vi "Measurement UI.vi"() -> ()   [LabVIEW 2021, in "Efficiency And Load Regulation_PMIC.lvlib"]
uses:
  Efficiency And Load Regulation_PMIC.lvlib
panel:
  in  "MeasGraphs":T1(tab)
  out "EfficiencyGraph":T2(graph)
  out "LoadRegulationGraph(V/A)":T2(graph)
  out "LoadRegulationGraph(%)":T2(graph)
  out "Maximum load regulation":dbl[](array[numeric])
  out "Minimum load regulation":dbl[](array[numeric])
  out "Maximum load voltage":dbl[](array[numeric])
  out "Minimum load voltage":dbl[](array[numeric])
  out "Maximum efficiency":dbl[](array[numeric])
  out "Minimum efficiency":dbl[](array[numeric])
  out "Source sweep points":i32
  out "Load voltage deviation":dbl[](array[numeric])
  out "Load voltages":dbl[](array[numeric])
  out "Voltage values":dbl[](array[numeric])
  out "Load sweep points":i32
  out "Efficiency":dbl[](array[numeric])
  out "Load currents":dbl[](array[numeric])
  in  "Source resource name":string caption="RESOURCE NAME"
  in  "Load resource name":string caption="RESOURCE NAME"
  out "MeasTable":string[][](table)
  in  "Measurement timeout":dbl=10.0 caption="MEASUREMENT TIME-OUT" format="%#_6ps"
  in  "Load sense":i32(ring)=1009 caption="SENSE" items=["Local"=1008, "Remote"=1009]
  in  "Source sense":i32(ring)=1009 caption="SENSE" items=["Local"=1008, "Remote"=1009]
  out "Status":string
  in  "ELOADResourceName":refnum<k15> caption="RESOURCE NAME"
  in  "PPSResourceName":refnum<k15> caption="RESOURCE NAME"
  in  "Load sweep type":string(combo)="Logarithmic" caption="SWEEP TYPE"
  in  "DUT setup time":dbl=1.0 caption="DUT SETUP TIME" format="%#_6ps"
  in  "Source stop voltage":dbl=20.0 caption="STOP VOLTAGE" format="%#_6pV"
  in  "Source start voltage":dbl=6.0 caption="START VOLTAGE" format="%#_6pV"
  in  "Source voltage sweep points":i32=4 caption="NO. OF POINTS"
  in  "Aperture time":dbl=0.005 caption="APERTURE TIME" format="%#_6ps"
  in  "Source delay":dbl=0.005 caption="SOURCE DELAY" format="%#_6ps"
  in  "Load current sweep points/points per decade":i32=10 caption="PTS/PTS PER DECADE"
  in  "Load stop current":dbl=24.0 caption="STOP CURRENT" format="%#_6pA"
  in  "Load start current":dbl=0.1 caption="START CURRENT" format="%#_6pA"
  in  "Load voltage limit range":dbl=6.0 caption="VOLTAGE LIMIT RANGE" format="%#_6pV"
  in  "Source current limit":dbl=25.0 caption="CURRENT LIMIT" format="%#_6pA"
  in  "Source maximum power":dbl=300.0 caption="MAXIMUM POWER" format="%#_6pW"
  in  "Load configuration":string="Load configuration"
  in  "Source configuration":string="Source configuration"
  in  "Measurement settings":string="Measurement settings"
  in  "Nominal output voltage":dbl=3.3 caption="NOMINAL OUTPUT VOLTAGE" format="%#_6pV"
  in  "Mode of operation":T3(ring)=enum."Perform measurement" caption="MODE OF OPERATION"
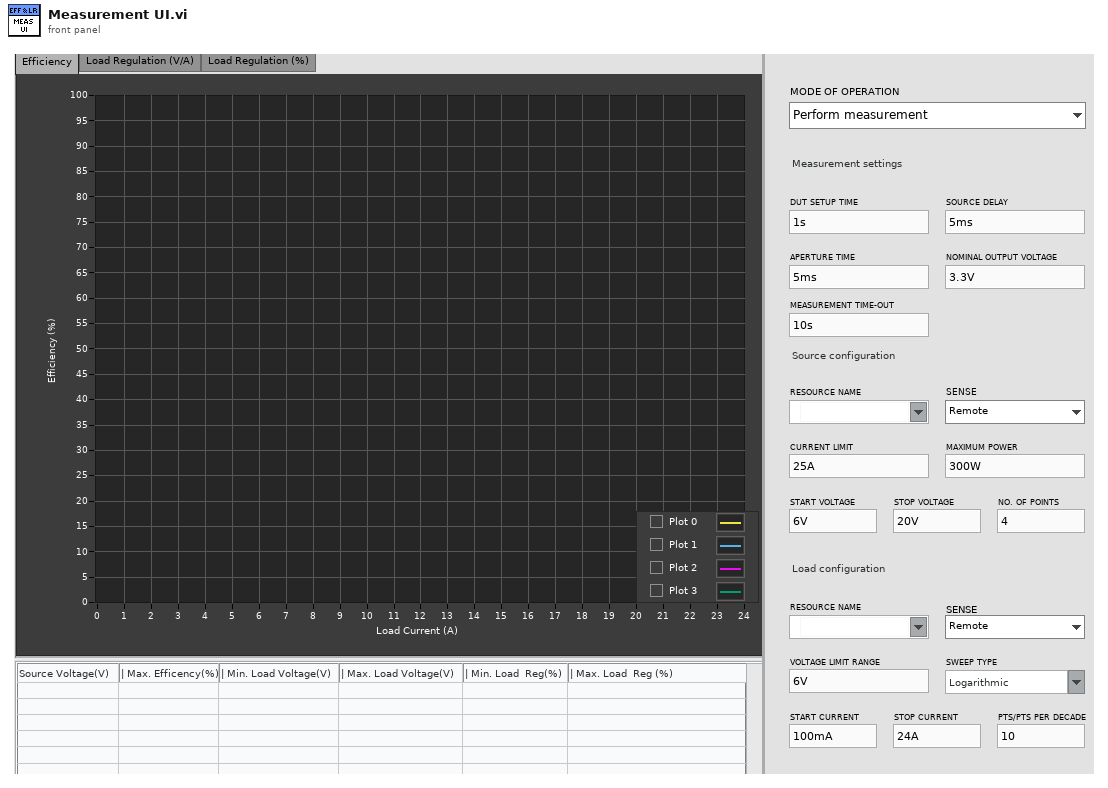
[diagram p1: front panel]
types:
  T1 = enum32{"Efficiency", "Load Regulation (V/A)", "Load Regulation (%)", "Hidden Controls"}
  T2 = cluster{"Load currents":dbl[], "Efficiency":dbl[]}[]
  T3 = enum32{"Power on the DUT", "Perform measurement", "Power off the DUT"}
  T4 = cluster{"Load currents":dbl[], "Efficiency":dbl[]}
  T5 = cluster{"Load currents":dbl[], "Load voltages":dbl[]}
  T6 = cluster{"Load currents":dbl[], "Load voltage deviation":dbl[]}
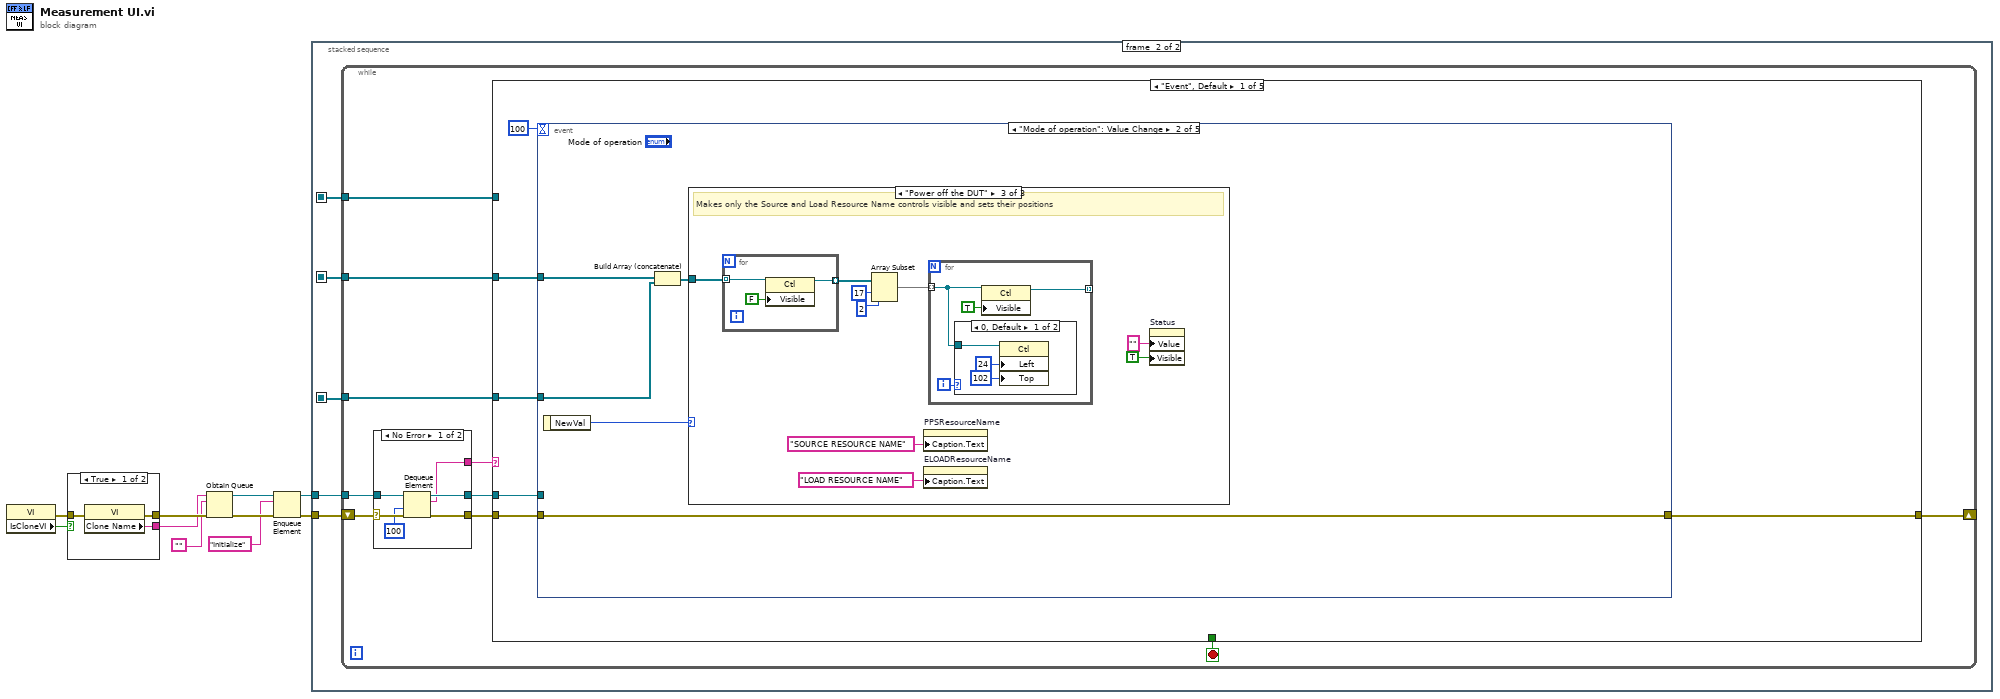
[diagram p0: block diagram]
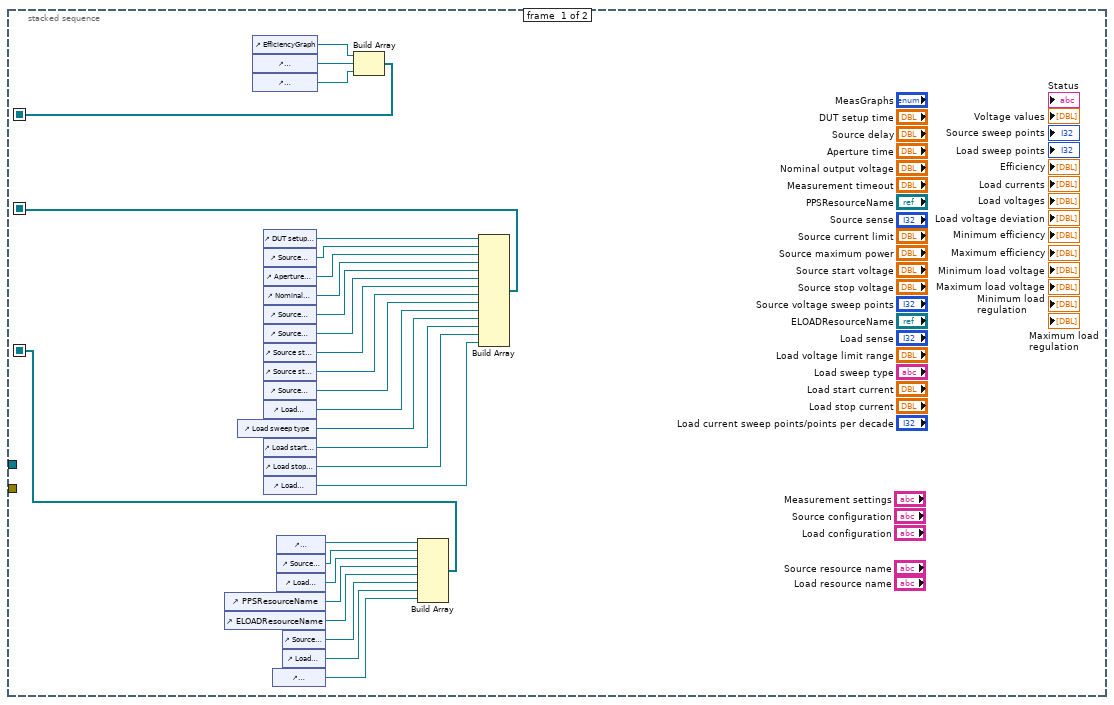
[diagram p2: hidden frame]
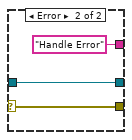
[diagram p3: hidden frame]
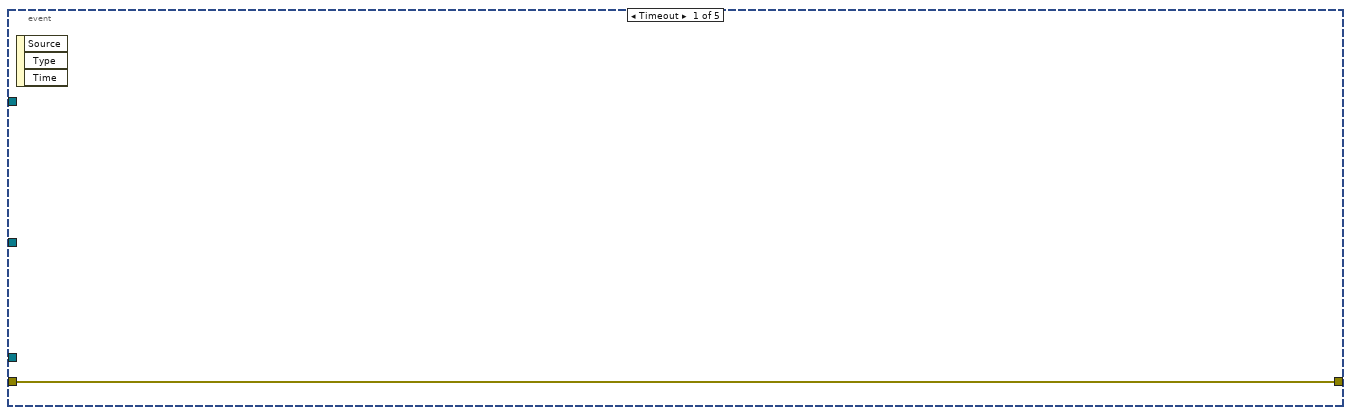
[diagram p4: hidden frame]
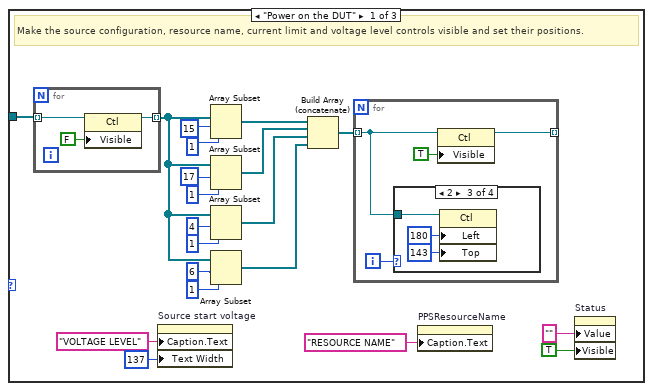
[diagram p5: hidden frame]
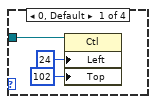
[diagram p6: hidden frame]
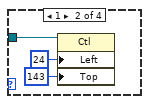
[diagram p7: hidden frame]
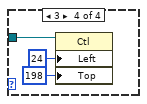
[diagram p8: hidden frame]
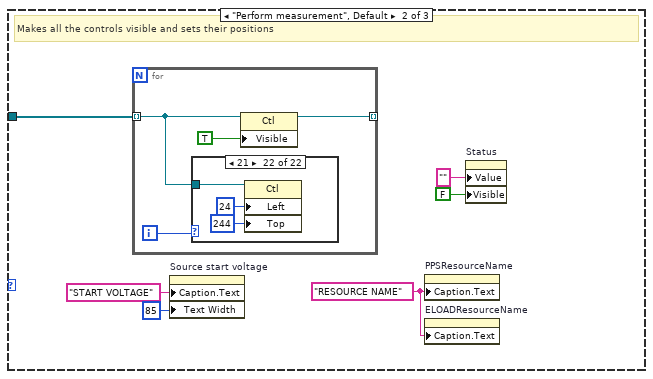
[diagram p9: hidden frame]
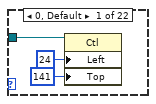
[diagram p10: hidden frame]
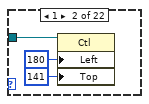
[diagram p11: hidden frame]
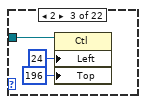
[diagram p12: hidden frame]
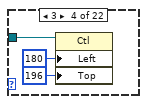
[diagram p13: hidden frame]
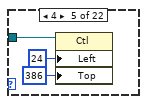
[diagram p14: hidden frame]
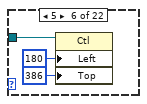
[diagram p15: hidden frame]
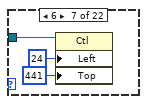
[diagram p16: hidden frame]
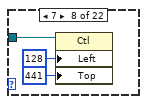
[diagram p17: hidden frame]
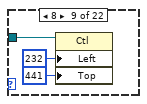
[diagram p18: hidden frame]
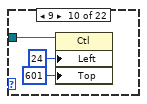
[diagram p19: hidden frame]
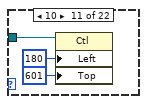
[diagram p20: hidden frame]
diagram:
  n1 = property class="VI"() -> (error out=w1:errorcluster, "IsCloneVI"=w2:bool)  [unwired: 2 in, 1 out]
  n2 = case shown="True" w2 {
    tunnel: [w13 w16] -> w10
    tunnel: [w12 w15] -> w9
    tunnel: w1 -> [w11 w14]
    frame True {
      n3 = property class="VI"(error in=w11) -> (error out=w13:errorcluster, "Clone Name"=w12:string)  [unwired: 1 in, 1 out]
    }
    frame False {
      n4 = property class="VI"(error in=w14) -> (error out=w16:errorcluster, "Name"=w15:string)  [unwired: 1 in, 1 out]
    }
  }
  n5 = Obtain Queue(name (unnamed)=w9, element data type="", error in (no error)=w10) -> (queue out=w6:refnum<queue>, error out=w8:errorcluster)  [unwired: 2 in, 1 out]
  n6 = Enqueue Element(queue=w6, element="Initialize", error in (no error)=w8) -> (queue out=w5:refnum<queue>, error out=w7:errorcluster)  [unwired: 1 in, 1 out]
  n7 = stacked-sequence {
    seq-local: [w20 _] -> [_ w47]
    seq-local: [w21 _] -> [_ w46]
    seq-local: [w22 _] -> [_ w45]
    tunnel: w7 -> [_ w49]
    tunnel: w5 -> [_ w48]
    frame #0 {
      n8 = control-ref of="PPSResourceName"() -> (w27:refnum<vi>)
      n9 = control-ref of="ELOADResourceName"() -> (w26:refnum<vi>)
      n10 = control-ref of="Load sweep type"() -> (w35:refnum<vi>)
      n11 = control-ref of="EfficiencyGraph"() -> (w25:refnum<vi>)
      n12 = control-ref of="LoadRegulationGraph(V/A)"() -> (w24:refnum<vi>)
      n13 = control-ref of="LoadRegulationGraph(%)"() -> (w23:refnum<vi>)
      n14 = control-ref of="DUT setup time"() -> (w44:refnum<vi>)
      n15 = control-ref of="Source delay"() -> (w43:refnum<vi>)
      n16 = control-ref of="Aperture time"() -> (w42:refnum<vi>)
      n17 = control-ref of="Nominal output voltage"() -> (w31:refnum<vi>)
      n18 = control-ref of="Source current limit"() -> (w41:refnum<vi>)
      n19 = control-ref of="Source maximum power"() -> (w40:refnum<vi>)
      n20 = control-ref of="Source start voltage"() -> (w39:refnum<vi>)
      n21 = control-ref of="Source stop voltage"() -> (w38:refnum<vi>)
      n22 = control-ref of="Source voltage sweep points"() -> (w37:refnum<vi>)
      n23 = control-ref of="Load voltage limit range"() -> (w36:refnum<vi>)
      n24 = control-ref of="Load start current"() -> (w34:refnum<vi>)
      n25 = control-ref of="Load stop current"() -> (w33:refnum<vi>)
      n26 = control-ref of="Load current sweep points/points per decade"() -> (w32:refnum<vi>)
      n27 = control-ref of="Measurement timeout"() -> (w17:refnum<vi>)
      n28 = control-ref of="Measurement settings"() -> (w30:refnum<vi>)
      n29 = control-ref of="Source configuration"() -> (w28:refnum<vi>)
      n30 = control-ref of="Load configuration"() -> (w29:refnum<vi>)
      n31 = control-ref of="Source sense"() -> (w19:refnum<vi>)
      n32 = control-ref of="Load sense"() -> (w18:refnum<vi>)
      n33 = Build Array(w25, w24, w23) -> (w20:refnum<vi>[])
      n34 = Build Array(w30, w28, w29, w27, w26, w19, w18, w17) -> (w22:refnum<vi>[])
      n35 = Build Array(w44, w43, w42, w31, w41, w40, w39, w38, w37, w36, w35, w34, w33, w32) -> (w21:refnum<vi>[])
    }
    frame #1 {
      n36 = while {
        shift-right: [w54] -> _
        shift-left: w49 -> [w59]
        tunnel: w48 -> [w57]
        tunnel: w46 -> [w52]
        tunnel: w45 -> [w51]
        tunnel: w47 -> [w50]
        stop <- w53 stop-if-true
        n37 = case shown="No Error" w59 {
          selector: w59 -> [w65 w68]
          tunnel: [w64 w68] -> w58
          tunnel: w57 -> [w63 w67]
          tunnel: [w62 w67] -> w56
          tunnel: [w61 "Handle Error"] -> w55
          frame No Error {
            n38 = Dequeue Element(queue=w63, timeout in ms (-1)=100, error in (no error)=w65) -> (queue out=w62:refnum<queue>, element=w61:string, error out=w64:errorcluster)  [unwired: 1 out]
          }
          frame Error {
          }
        }
        n39 = case shown="\"Event\", Default" w55 {
          tunnel: w58 -> [w73 w230 w253 w331 w332]
          tunnel: w56 -> [w71 _ _ w329 _]
          tunnel: [w74 w230 w253 w323 w332] -> w54
          tunnel: [_ _ _ TRUE _] -> w53
          tunnel: w52 -> [w70 _ _ w321 _]
          tunnel: w51 -> [w69 _ _ w320 _]
          tunnel: w50 -> [_ w229 w243 w322 _]
          frame "Event", Default {
            n40 = event shown="[1] \"Mode of operation\": Value Change" {
              selector: _ -> [_ _ _ _ _]
              dyn-events: _ -> [_ _ _ _ _]
              timeout: 100 -> [_ _ _ _ _]
              tunnel: [w75 w76 w218 w220 w224] -> w74
              tunnel: w73 -> [w75 w76 w218 w220 w225]
              tunnel: w71 -> [_ _ _ _ w223]
              tunnel: w70 -> [_ w77 _ _ _]
              tunnel: w69 -> [_ w79 _ _ _]
              event Timeout {
                n41 = event-data() -> ()  [unwired: 1 in, 3 out]
              }
              event "Mode of operation": Value Change {
                n42 = event-data() -> ("NewVal"=w80:T3)  [unwired: 1 in]
                n43 = Build Array (concatenate)(w77, w79) -> (w78:refnum<vi>[])
                n44 = case shown="\"Power off the DUT\"" w80 {
                  tunnel: w78 -> [w92 w125 w201]
                  frame "Power on the DUT" {
                    # "Make the source configuration, resource name, current limit and voltage level controls visible and set their positions."
                    n45 = for {
                      tunnel: w92 -> [w103] mode=indexing
                      tunnel: [w101] -> w89 mode=indexing
                      n46 = property class="Ctl"(reference=w103, "Visible"=FALSE) -> (reference out=w101:refnum<vi>)  [unwired: 1 in, 1 out]
                    }
                    n47 = property on="Source start voltage" class="DigNum (strict)"("Caption.Text"="VOLTAGE LEVEL", "Text Width"=u32 137) -> ()  [unwired: 2 in, 2 out]
                    n48 = Array Subset(array=w89, index=15 ("length"), length=1 ("index")) -> (w91:refnum<vi>[])
                    n49 = Array Subset(array=w89, index=17 ("length"), length=1 ("index")) -> (w90:refnum<vi>[])
                    n50 = Array Subset(array=w89, index=4 ("length"), length=1 ("index")) -> (w88:refnum<vi>[])
                    n51 = Array Subset(array=w89, index=6 ("length"), length=1 ("index")) -> (w86:refnum<vi>[])
                    n52 = Build Array (concatenate)(w91, w90, w88, w86) -> (w87:refnum<vi>[])
                    n53 = for {
                      tunnel: [w106] -> _ mode=indexing
                      tunnel: w87 -> [w104] mode=indexing
                      i -> [w105]
                      n54 = case shown="2" w105 {
                        tunnel: w104 -> [w110 w113 w116 w119]
                        frame 0, Default {
                          n55 = property class="Ctl"(reference=w110, "Left"=24 ("Position:Left"), "Top"=102 ("Position:Top")) -> ()  [unwired: 1 in, 2 out]
                        }
                        frame 1 {
                          n56 = property class="Ctl"(reference=w113, "Left"=24 ("Position:Left"), "Top"=143 ("Position:Top")) -> ()  [unwired: 1 in, 2 out]
                        }
                        frame 2 {
                          n57 = property class="Ctl"(reference=w116, "Left"=180 ("Position:Left"), "Top"=143 ("Position:Top")) -> ()  [unwired: 1 in, 2 out]
                        }
                        frame 3 {
                          n58 = property class="Ctl"(reference=w119, "Left"=24 ("Position:Left"), "Top"=198 ("Position:Top")) -> ()  [unwired: 1 in, 2 out]
                        }
                      }
                      n59 = property class="Ctl"(reference=w104, "Visible"=TRUE) -> (reference out=w106:refnum<vi>)  [unwired: 1 in, 1 out]
                    }
                    n60 = property on="PPSResourceName" class="IVIName"("Caption.Text"="RESOURCE NAME") -> ()  [unwired: 2 in, 2 out]
                    n61 = property on="Status" class="Str"("Value"="" ("Status"), "Visible"=TRUE) -> ()  [unwired: 2 in, 2 out]
                  }
                  frame "Perform measurement", Default {
                    w123 = "RESOURCE NAME" ("Caption.Text")
                    # "Makes all the controls visible and sets their positions"
                    n62 = for {
                      tunnel: w125 -> [w126] mode=indexing
                      tunnel: [w128] -> _ mode=indexing
                      i -> [w127]
                      n63 = case shown="21" w127 {
                        tunnel: w126 -> [w132 w135 w138 w141 w144 w147 w150 w153 w156 w159 w162 w165 w168 w171 w174 w177 w180 w183 w186 w187 w190 w193]
                        frame 0, Default {
                          n64 = property class="Ctl"(reference=w132, "Left"=24 ("Position:Left"), "Top"=141 ("Position:Top")) -> ()  [unwired: 1 in, 2 out]
                        }
                        frame 1 {
                          n65 = property class="Ctl"(reference=w135, "Left"=180 ("Position:Left"), "Top"=141 ("Position:Top")) -> ()  [unwired: 1 in, 2 out]
                        }
                        frame 2 {
                          n66 = property class="Ctl"(reference=w138, "Left"=24 ("Position:Left"), "Top"=196 ("Position:Top")) -> ()  [unwired: 1 in, 2 out]
                        }
                        frame 3 {
                          n67 = property class="Ctl"(reference=w141, "Left"=180 ("Position:Left"), "Top"=196 ("Position:Top")) -> ()  [unwired: 1 in, 2 out]
                        }
                        frame 4 {
                          n68 = property class="Ctl"(reference=w144, "Left"=24 ("Position:Left"), "Top"=386 ("Position:Top")) -> ()  [unwired: 1 in, 2 out]
                        }
                        frame 5 {
                          n69 = property class="Ctl"(reference=w147, "Left"=180 ("Position:Left"), "Top"=386 ("Position:Top")) -> ()  [unwired: 1 in, 2 out]
                        }
                        frame 6 {
                          n70 = property class="Ctl"(reference=w150, "Left"=24 ("Position:Left"), "Top"=441 ("Position:Top")) -> ()  [unwired: 1 in, 2 out]
                        }
                        frame 7 {
                          n71 = property class="Ctl"(reference=w153, "Left"=128 ("Position:Left"), "Top"=441 ("Position:Top")) -> ()  [unwired: 1 in, 2 out]
                        }
                        frame 8 {
                          n72 = property class="Ctl"(reference=w156, "Left"=232 ("Position:Left"), "Top"=441 ("Position:Top")) -> ()  [unwired: 1 in, 2 out]
                        }
                        frame 9 {
                          n73 = property class="Ctl"(reference=w159, "Left"=24 ("Position:Left"), "Top"=601 ("Position:Top")) -> ()  [unwired: 1 in, 2 out]
                        }
                        frame 10 {
                          n74 = property class="Ctl"(reference=w162, "Left"=180 ("Position:Left"), "Top"=601 ("Position:Top")) -> ()  [unwired: 1 in, 2 out]
                        }
                        frame 11 {
                          n75 = property class="Ctl"(reference=w165, "Left"=24 ("Position:Left"), "Top"=656 ("Position:Top")) -> ()  [unwired: 1 in, 2 out]
                        }
                        frame 12 {
                          n76 = property class="Ctl"(reference=w168, "Left"=128 ("Position:Left"), "Top"=656 ("Position:Top")) -> ()  [unwired: 1 in, 2 out]
                        }
                        frame 13 {
                          n77 = property class="Ctl"(reference=w171, "Left"=232 ("Position:Left"), "Top"=656 ("Position:Top")) -> ()  [unwired: 1 in, 2 out]
                        }
                        frame 14 {
                          n78 = property class="Ctl"(reference=w174, "Left"=24 ("Position:Left"), "Top"=100 ("Position:Top")) -> ()  [unwired: 1 in, 2 out]
                        }
                        frame 15 {
                          n79 = property class="Ctl"(reference=w177, "Left"=24 ("Position:Left"), "Top"=292 ("Position:Top")) -> ()  [unwired: 1 in, 2 out]
                        }
                        frame 16 {
                          n80 = property class="Ctl"(reference=w180, "Left"=24 ("Position:Left"), "Top"=505 ("Position:Top")) -> ()  [unwired: 1 in, 2 out]
                        }
                        frame 17 {
                          n81 = property class="Ctl"(reference=w183, "Left"=24 ("Position:Left"), "Top"=331 ("Position:Top")) -> ()  [unwired: 1 in, 2 out]
                        }
                        frame 18 {
                          n82 = property class="Ctl"(reference=w186, "Left"=24 ("Position:Left"), "Top"=546 ("Position:Top")) -> ()  [unwired: 1 in, 2 out]
                        }
                        frame 19 {
                          n83 = property class="Ctl"(reference=w187, "Left"=180 ("Position:Left"), "Top"=331 ("Position:Top")) -> ()  [unwired: 1 in, 2 out]
                        }
                        frame 20 {
                          n84 = property class="Ctl"(reference=w190, "Left"=180 ("Position:Left"), "Top"=546 ("Position:Top")) -> ()  [unwired: 1 in, 2 out]
                        }
                        frame 21 {
                          n85 = property class="Ctl"(reference=w193, "Left"=24 ("Position:Left"), "Top"=244 ("Position:Top")) -> ()  [unwired: 1 in, 2 out]
                        }
                      }
                      n86 = property class="Ctl"(reference=w126, "Visible"=TRUE) -> (reference out=w128:refnum<vi>)  [unwired: 1 in, 1 out]
                    }
                    n87 = property on="Source start voltage" class="DigNum (strict)"("Caption.Text"="START VOLTAGE", "Text Width"=u32 85) -> ()  [unwired: 2 in, 2 out]
                    n88 = property on="PPSResourceName" class="IVIName"("Caption.Text"=w123) -> ()  [unwired: 2 in, 2 out]
                    n89 = property on="ELOADResourceName" class="IVIName"("Caption.Text"=w123) -> ()  [unwired: 2 in, 2 out]
                    n90 = property on="Status" class="Str"("Value"="" ("Status"), "Visible"=FALSE) -> ()  [unwired: 2 in, 2 out]
                  }
                  frame "Power off the DUT" {
                    # "Makes only the Source and Load Resource Name controls visible and sets their positions"
                    n91 = for {
                      tunnel: w201 -> [w206] mode=indexing
                      tunnel: [w205] -> w200 mode=indexing
                      n92 = property class="Ctl"(reference=w206, "Visible"=FALSE) -> (reference out=w205:refnum<vi>)  [unwired: 1 in, 1 out]
                    }
                    n93 = Array Subset(array=w200, index=17 ("length"), length=2 ("index")) -> (w202:refnum<vi>[])
                    n94 = property on="PPSResourceName" class="IVIName"("Caption.Text"="SOURCE RESOURCE NAME") -> ()  [unwired: 2 in, 2 out]
                    n95 = property on="ELOADResourceName" class="IVIName"("Caption.Text"="LOAD RESOURCE NAME") -> ()  [unwired: 2 in, 2 out]
                    n96 = for {
                      tunnel: w202 -> [w208] mode=indexing
                      tunnel: [w210] -> _ mode=indexing
                      i -> [w209]
                      n97 = case shown="0, Default" w209 {
                        tunnel: w208 -> [w214 w217]
                        frame 0, Default {
                          n98 = property class="Ctl"(reference=w214, "Left"=24 ("Position:Left"), "Top"=102 ("Position:Top")) -> ()  [unwired: 1 in, 2 out]
                        }
                        frame 1 {
                          n99 = property class="Ctl"(reference=w217, "Left"=24 ("Position:Left"), "Top"=157 ("Position:Top")) -> ()  [unwired: 1 in, 2 out]
                        }
                      }
                      n100 = property class="Ctl"(reference=w208, "Visible"=TRUE) -> (reference out=w210:refnum<vi>)  [unwired: 1 in, 1 out]
                    }
                    n101 = property on="Status" class="Str"("Value"="" ("Status"), "Visible"=TRUE) -> ()  [unwired: 2 in, 2 out]
                  }
                }
              }
              event "PPSResourceName": Value Change {
                n102 = event-data() -> ()  [unwired: 1 in, 1 out]
                n103 = property on="PPSResourceName" class="IVIName"() -> ("Value"=w219:refnum<k15>)  [unwired: 2 in, 2 out]
                n104 = property on="Source resource name" class="Str"("Value"=w219) -> ()  [unwired: 2 in, 2 out]
              }
              event "ELOADResourceName": Value Change {
                n105 = event-data() -> ()  [unwired: 1 in, 1 out]
                n106 = property on="ELOADResourceName" class="IVIName"() -> ("Value"=w221:refnum<k15>)  [unwired: 2 in, 2 out]
                n107 = property on="Load resource name" class="Str"("Value"=w221) -> ()  [unwired: 2 in, 2 out]
              }
              event Panel Close? {
                n108 = event-data() -> ()  [unwired: 1 in, 4 out]
                n109 = Enqueue Element(queue=w223, element="Exit", error in (no error)=w225) -> (error out=w224:errorcluster)  [unwired: 1 in, 2 out]
                n110 = event-data("Discard?"=TRUE) -> ()  [unwired: 1 in, 1 out]
              }
            }
          }
          frame "Initialize" {
            w228 = "<Select Device>"
            n111 = for {
              tunnel: w229 -> [w231] mode=indexing
              n112 = property class="XYGraph (strict)"(reference=w231, "ActPaletteTool"=2 ("Palette:Active Tool")) -> ()  [unwired: 1 in, 2 out]
            }
            n113 = property on="PPSResourceName" class="IVIName"("Value"=w228) -> ()  [unwired: 2 in, 2 out]
            n114 = property on="ELOADResourceName" class="IVIName"("Value"=w228) -> ()  [unwired: 2 in, 2 out]
            n115 = property on="Status" class="Str"("Visible"=FALSE) -> ()  [unwired: 2 in, 2 out]
          }
          frame "Post UI Update" {
            w242 = u32[] [15787074, 5682409, 15535092, 40563, 13983232, 35009, 15113984, 13400487, 15993633, 10221451, 8148942, 15869817, 32914, 10196480, 6271923, 16355671]  # Plot colors
            # "-Sets various properties of graphs like color, point style, plot name etc.\n-Increases the legend number of rows if the voltage values are less than 4 and \nif it is greater than 4 then make the default rows as 4 and enable the vertical scrollbar.\n-Also sets the plot minimum property to source sweep points which disables the unused plots in the graph."
            # "Plot the deleted array in the graph"
            # "This case will be triggered, after framework updates the User interface with result values."
            n116 = local read "Source sweep points"() -> (w241:i32)
            n117 = local read "Voltage values"() -> (w239:dbl[])
            n118 = for {
              tunnel: w239 -> [w273]
              tunnel: [w272] -> w240
              tunnel: w243 -> [w271] mode=indexing
              tunnel: w241 -> [w270]
              tunnel: w242 -> [w269]
              n119 = for {
                tunnel: w273 -> [w286] mode=indexing
                tunnel: [w286] -> w272 mode=indexing
                tunnel: w271 -> [w279]
                tunnel: w270 -> [w276]
                tunnel: w269 -> [w282] mode=indexing
                i -> [w280]
                n120 = Greater?(x=w280, y=3) -> (0:w284:bool)
                n121 = To Unsigned Long Integer(number=w280) -> (unsigned 32bit integer=w283:u32)
                n122 = Increment(x=w280) -> (x+1=w278:i32)
                n123 = Format Value(format string="%.3f", value (0)=w286) -> (output string=w289:string)  [unwired: 1 out]
                n124 = case shown="False" w284 {
                  tunnel: w279 -> [w295 w301]
                  tunnel: w278 -> [w294 _]
                  tunnel: [w293 w300] -> w277
                  tunnel: w276 -> [w291 w296]
                  tunnel: [w292 w299] -> w275
                  frame False {
                    n125 = property on="Property Node" class="XYGraph (strict)"(reference=w295, "LegScrollVis"=FALSE ("Legend:Scrollbar Visible"), "LegNumRows"=w294, "LegPlotMin"=w291) -> (reference out=w293:refnum<vi>, error out=w292:errorcluster)  [unwired: 1 in]
                  }
                  frame True {
                    n126 = property on="Property Node" class="XYGraph (strict)"(reference=w301, "LegScrollVis"=TRUE ("Legend:Scrollbar Visible"), "LegNumRows"=u32 4 ("Legend:Number of Rows"), "LegPlotMin"=w296) -> (reference out=w300:refnum<vi>, error out=w299:errorcluster)  [unwired: 1 in]
                  }
                }
                n127 = Concatenate Strings(" Vin = " ("string"), w289) -> (w274:string)
                n128 = property on="Property Node" class="XYGraph (strict)"(reference=w277, error in=w275, "Active Plot"=w283, "Plot.Point Style"=u8 5, "Plot.Plot Color"=w282, "Plot.Fill/Pt. Color"=w282, "Plot.Plot Name"=w274) -> ()  [unwired: 2 out]
              }
            }
            n129 = local read "Maximum load regulation"() -> (w234:dbl[])
            n130 = local read "Minimum load regulation"() -> (w235:dbl[])
            n131 = local read "Maximum load voltage"() -> (w236:dbl[])
            n132 = local read "Minimum load voltage"() -> (w237:dbl[])
            n133 = local read "Maximum efficiency"() -> (w238:dbl[])
            n134 = Array Size(array=w240) -> (size(s)=w250:i32)
            n135 = local read "Load voltage deviation"() -> (w252:dbl[])
            n136 = local read "Load sweep points"() -> (w247:i32)
            n137 = local read "Load voltages"() -> (w251:dbl[])
            n138 = local read "Load currents"() -> (w249:dbl[])
            n139 = local read "Efficiency"() -> (w248:dbl[])
            n140 = for {
              N: w250 -> [_]
              tunnel: [w318] -> w244 mode=indexing
              tunnel: [w317] -> w245 mode=indexing
              tunnel: [w316] -> w246 mode=indexing
              tunnel: w247 -> [w303]
              shift-right: [w311] -> _
              shift-left: w249 -> [w315]
              shift-right: [w309] -> _
              shift-left: w248 -> [w314]
              shift-right: [w308] -> _
              shift-left: w251 -> [w313]
              shift-right: [w307] -> _
              shift-left: w252 -> [w312]
              w302 = 0 ("index")
              n141 = Delete From Array(array=w315, length=w303, index=w302) -> (deleted portion=w310:dbl[], array with subset deleted=w311:dbl[])
              n142 = Delete From Array(array=w314, length=w303, index=w302) -> (deleted portion=w304:dbl[], array with subset deleted=w309:dbl[])
              n143 = Delete From Array(array=w313, length=w303, index=w302) -> (deleted portion=w305:dbl[], array with subset deleted=w308:dbl[])
              n144 = Delete From Array(array=w312, length=w303, index=w302) -> (deleted portion=w306:dbl[], array with subset deleted=w307:dbl[])
              n145 = Bundle("Load currents"=w310, "Efficiency"=w304) -> (w318:T4)  [unwired: 1 in]
              n146 = Bundle("Load currents"=w310, "Load voltages"=w305) -> (w317:T5)  [unwired: 1 in]
              n147 = Bundle("Load currents"=w310, "Load voltage deviation"=w306) -> (w316:T6)  [unwired: 1 in]
            }
            "EfficiencyGraph" <- w244
            "LoadRegulationGraph(V/A)" <- w245
            "LoadRegulationGraph(%)" <- w246
            n148 = for {
              tunnel: w237 -> [w266] mode=indexing
              tunnel: [w268] -> w233 mode=indexing
              tunnel: w238 -> [w267] mode=indexing
              tunnel: w236 -> [w265] mode=indexing
              tunnel: w235 -> [w264] mode=indexing
              tunnel: w239 -> [w260] mode=indexing
              tunnel: w234 -> [w255] mode=indexing
              w257 = "%0.9f" ("initial string")
              w256 = "| " ("initial string")
              n149 = Format Into String(format string=w257, w260) -> (resulting string=w259:string)  [unwired: 2 in, 1 out]
              n150 = Format Into String(format string=w257, initial string=w256, w267) -> (resulting string=w263:string)  [unwired: 1 in, 1 out]
              n151 = Format Into String(format string=w257, initial string=w256, w266) -> (resulting string=w262:string)  [unwired: 1 in, 1 out]
              n152 = Format Into String(format string=w257, initial string=w256, w265) -> (resulting string=w261:string)  [unwired: 1 in, 1 out]
              n153 = Format Into String(format string=w257, initial string=w256, w264) -> (resulting string=w258:string)  [unwired: 1 in, 1 out]
              n154 = Format Into String(format string=w257, initial string=w256, w255) -> (resulting string=w254:string)  [unwired: 1 in, 1 out]
              n155 = Build Array(w259, w263, w262, w261, w258, w254) -> (w268:string[])
            }
            "MeasTable" <- w233
          }
          frame "Exit" {
            # "This case is triggered to close the User Interface from framework"
            n156 = Build Array (concatenate)(w322, w321, w320) -> (w319:refnum<vi>[])
            n157 = Close Reference(reference=w319) -> (error out=w325:errorcluster)  [unwired: 1 in]
            n158 = Flush Queue(queue=w329, error in (no error)=w331) -> (queue out=w328:refnum<queue>, error out=w327:errorcluster)  [unwired: 1 out]
            n159 = Release Queue(queue=w328, force destroy? (F)=TRUE, error in (no error)=w327) -> (error out=w324:errorcluster)  [unwired: 2 out]
            n160 = Merge Errors(w325, w324) -> (w323:errorcluster)
          }
          frame "Handle Error" {
          }
        }
      }
    }
  }
